vi "Main.vi"() -> ()   [LabVIEW 2018, in "BridgePatternDemo.lvclass"]
uses:
  BridgePatternDemo.lvclass
  Tv Class/Tv.lvclass
  C:/Users/fflores/Documents/LabVIEW-Open-Projects/LabIVEW OOP Design Patterns/Bridge Pattern/Device Class/Device.lvclass
  Radio Class/Radio.lvclass
  ConsoleOut/Print Options.ctl
panel:
  out "error out":errorcluster
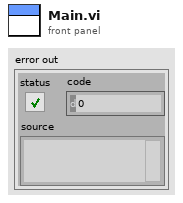
[diagram p1: front panel]
types:
  T1 = typedef "Print Options.ctl" = enum16{"Create", "Get Reference", "Print", "Print Header", "Close"}
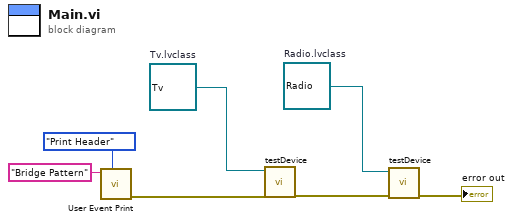
[diagram p0: block diagram]
diagram:
  w5 = refnum<class "Radio.lvclass"> refnum  # Radio.lvclass
  w7 = refnum<class "Tv.lvclass"> refnum  # Tv.lvclass
  n1 = call "User Event Print.vi"("Options"=Print_Options."Print Header", "String to Print"="Bridge Pattern") -> ("error out"=w4:errorcluster)  [unwired: 8 in, 1 out]
  n2 = call "testDevice.vi"("error in (no error)"=w4, "Device.lvclass"=w7) -> ("error out"=w6:errorcluster)  [unwired: 9 in]
  n3 = call "testDevice.vi"("error in (no error)"=w6, "Device.lvclass"=w5) -> ("error out"=→"error out":errorcluster)  [unwired: 9 in]
